vi "measure PSD Trace Values Type using CSV File.vi"(8 "error in (no error)":errorcluster, 11 "SA Measurement in":refnum<class "SA Measurement.lvclass">) -> (0 "error out":errorcluster, 3 "SA Measurement out":refnum<class "SA Measurement.lvclass">)   [LabVIEW 2023, in "Spectrum Analyzer.lvlib" / "SA Measurement.lvclass"]
uses:
  SA Measurement.lvclass
  SA Measurement.lvclass/SA Measurement.ctl
  TYPE DEFINITION/Keysight 9020A/TYPE Measurement Preset.ctl
  Spectrum Analyzer.lvlib
  TYPE DEFINITION/TYPE RBW and VBW Select.ctl
  Interface_Spectrum/Interface_Spectrum.lvclass
  TYPE DEFINITION/TYPE Marker Peak Search Type.ctl
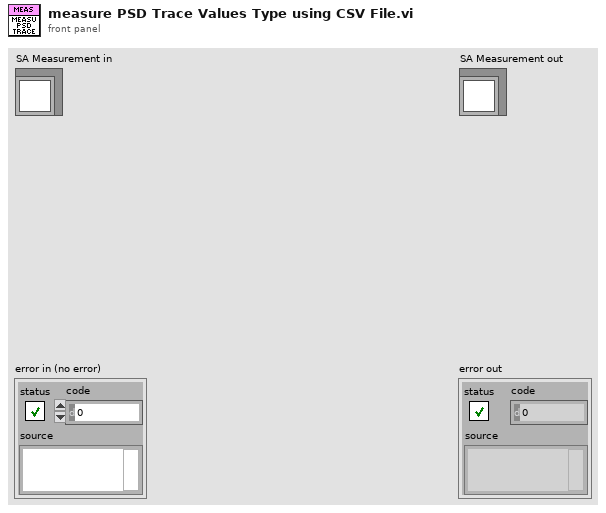
[diagram p1: front panel]
types:
  T1 = typedef "Spectrum Analyzer.lvlib/TYPE Marker Peak Search Type.ctl" = enum16{"Max", "Next Peak"}
  T2 = typedef "Spectrum Analyzer.lvlib/TYPE RBW and VBW Select.ctl" = enum16{"Res BW", "Video BW"}
  T3 = typedef "Spectrum Analyzer.lvlib/TYPE Measurement Preset.ctl" = enum16{"Sweep SA Mode", "Channel Power", "Occupied BW", "ACP", "Spurious Emission", "Spurious Emission Mask", "Burst Power (Transmit Power)"}
  T4 = typedef "Spectrum Analyzer.lvlib/TYPE Y-axis Unit.ctl" = enum16{"dBm", "dBmV", "dBuV", "dBpW", "Volt", "Ampere", "Watt"}
  T5 = typedef "Spectrum Analyzer.lvlib/TYPE Reference Level and Atten Param.ctl" = cluster{"Reference Level":dbl, "Atten":i32, "Atten Auto?":bool, "Reference Level Offset":dbl}
  T6 = typedef "Spectrum Analyzer.lvlib/TYPE Start and Stop Frequency.ctl" = cluster{"Start":dbl, "Stop":dbl}
  T7 = typedef "Spectrum Analyzer.lvlib/TYPE Display Trace Mode Select.ctl" = enum16{"Clear Write", "Max Hold", "Min Hold", "Average", "View"}
  T8 = typedef "Spectrum Analyzer.lvlib/TYPE Detect Mode Select.ctl" = enum16{"Det Auto (Normal)", "Auto Peak", "Positive Peak", "Negative Peak", "Sample", "RMS", "Average", "Quasipeak", "CISPR Average", "RMS Average"}
  T9 = cluster{"Trace Mode":T7, "Detector Type":T8, "Detect Auto?":bool}[]
  T10 = typedef "Spectrum Analyzer.lvlib/TYPE Average Mode Select.ctl" = enum16{"Linear(Voltage Avg)", "Video(Log)", "Power"}
  T11 = typedef "Spectrum Analyzer.lvlib/TYPE Marker Value.ctl" = cluster{"X-axis":dbl, "Y-axis":dbl}
  T12 = typedef "Spectrum Analyzer.lvlib/TYPE Trace Value Array.ctl" = cluster{"Frequency":dbl[], "Amplitude":dbl[]}
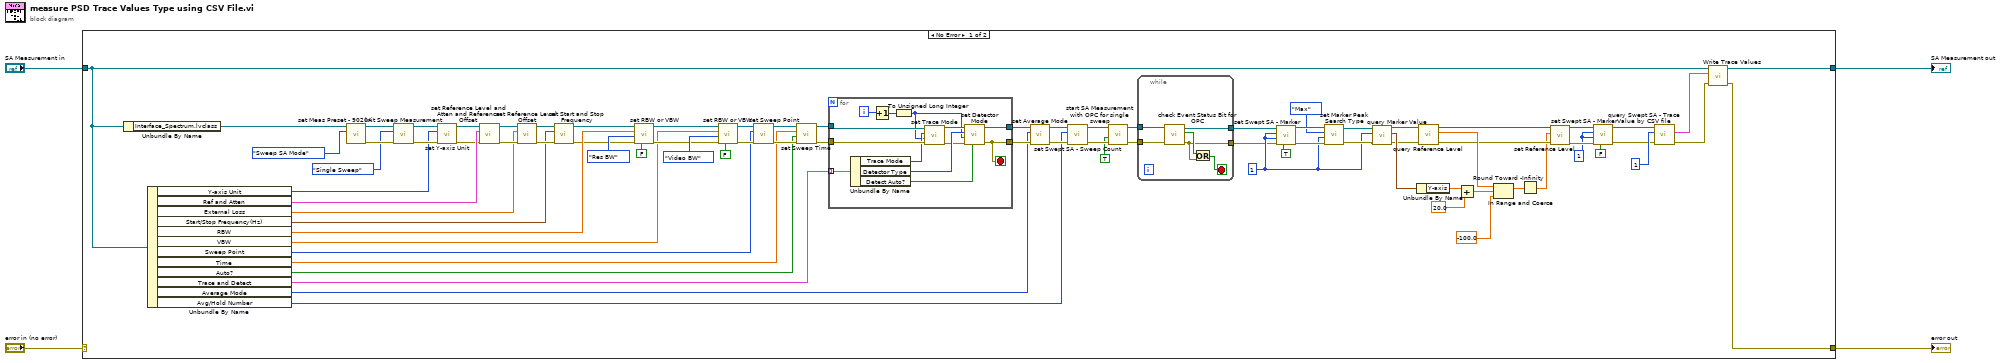
[diagram p0: block diagram]
diagram:
  n1 = case shown="No Error" "error in (no error)" {
    selector: "error in (no error)" -> [_ w106]
    tunnel: [w35 w106] -> w3
    tunnel: [w36 w105] -> w1
    tunnel: "SA Measurement in" -> [w37 w105]
    frame No Error {
      w12 = 1 ("Index")
      w28 = 1 ("Index")
      n2 = Unbundle By Name(w37) -> ("Interface_Spectrum.lvclass"=w85:refnum<class "Interface_Spectrum.lvclass">)
      n3 = Unbundle By Name(w37) -> ("Y-axis Unit"=w64:T4, "Ref and Atten"=w80:T5, "External Loss"=w77:dbl, "Start/Stop Frequency(Hz)"=w39:T6, "RBW"=w76:dbl, "VBW"=w69:dbl, "Sweep Point"=w61:u32, "Time"=w58:dbl, "Auto?"=w57:bool, "Trace and Detect"=w54:T9, "Average Mode"=w51:T10, "Avg/Hold Number"=w48:u32)
      n4 = call-dynamic "set Meas Preset - 9020A.vi"("Measurement Preset"=TYPE_Measurement_Preset."Sweep SA Mode", "Interface_Spectrum in"=w85) -> ("error out"=w82:errorcluster, "Interface_Spectrum out"=w83:refnum<class "Interface_Spectrum.lvclass">)  [unwired: 8 in]
      n5 = call-dynamic "init Sweep Measurement.vi"("error in (no error)"=w82, "Sweep Measurement Mode"=enum16{"Single Sweep", "Continuous Sweep"}."Single Sweep", "Interface_Spectrum in"=w83) -> ("error out"=w67:errorcluster, "Interface_Spectrum out"=w68:refnum<class "Interface_Spectrum.lvclass">)  [unwired: 7 in]
      n6 = call-dynamic "set Y-axis Unit.vi"("error in (no error)"=w67, "Y-axis Unit"=w64, "Interface_Spectrum in"=w68) -> ("error out"=w65:errorcluster, "Interface_Spectrum out"=w66:refnum<class "Interface_Spectrum.lvclass">)  [unwired: 7 in]
      n7 = call-dynamic "set Reference Level and Atten and Reference Offset.vi"("error in (no error)"=w65, "Reference Level, Atten, Reference Offset"=w80, "Interface_Spectrum in"=w66) -> ("error out"=w78:errorcluster, "Interface_Spectrum out"=w79:refnum<class "Interface_Spectrum.lvclass">)  [unwired: 7 in]
      n8 = call-dynamic "set Reference Level Offset.vi"("error in (no error)"=w78, "Reference Level Offset"=w77, "Interface_Spectrum in"=w79) -> ("error out"=w40:errorcluster, "Interface_Spectrum out"=w42:refnum<class "Interface_Spectrum.lvclass">)  [unwired: 7 in]
      n9 = call-dynamic "set Start and Stop Frequency.vi"("error in (no error)"=w40, "Start/Stop Frequency(Hz)"=w39, "Interface_Spectrum in"=w42) -> ("error out"=w38:errorcluster, "Interface_Spectrum out"=w41:refnum<class "Interface_Spectrum.lvclass">)  [unwired: 7 in]
      n10 = call-dynamic "set RBW or VBW.vi"("BW Auto?"=FALSE, "error in (no error)"=w38, "BW Type"=TYPE_RBW_and_VBW_Select."Res BW", "BW Value (Hz)"=w76, "Interface_Spectrum in"=w41) -> ("error out"=w70:errorcluster, "Interface_Spectrum out"=w71:refnum<class "Interface_Spectrum.lvclass">)  [unwired: 5 in]
      n11 = call-dynamic "set RBW or VBW.vi"("BW Auto?"=FALSE, "error in (no error)"=w70, "BW Type"=TYPE_RBW_and_VBW_Select."Video BW", "BW Value (Hz)"=w69, "Interface_Spectrum in"=w71) -> ("error out"=w62:errorcluster, "Interface_Spectrum out"=w63:refnum<class "Interface_Spectrum.lvclass">)  [unwired: 5 in]
      n12 = call-dynamic "set Sweep Point.vi"("error in (no error)"=w62, "Sweep Point"=w61, "Interface_Spectrum in"=w63) -> ("error out"=w59:errorcluster, "Interface_Spectrum out"=w60:refnum<class "Interface_Spectrum.lvclass">)  [unwired: 7 in]
      n13 = call-dynamic "set Sweep Time.vi"("error in (no error)"=w59, "Sweep Time Auto?"=w57, "Sweep Time(sec)"=w58, "Interface_Spectrum in"=w60) -> ("error out"=w55:errorcluster, "Interface_Spectrum out"=w56:refnum<class "Interface_Spectrum.lvclass">)  [unwired: 6 in]
      n14 = for {
        tunnel: w56 -> [w103]
        tunnel: w55 -> [w102]
        tunnel: w54 -> [w104] mode=indexing
        tunnel: [w92] -> w52
        tunnel: [w93] -> w53
        i -> [w101]
        stop <- w92 stop-if-true
        n15 = Unbundle By Name(w104) -> ("Trace Mode"=w99:T7, "Detector Type"=w97:T8, "Detect Auto?"=w94:bool)
        n16 = Increment(x=w101) -> (x+1=w100:i32)
        n17 = To Unsigned Long Integer(number=w100) -> (unsigned 32bit integer=w95:u32)
        n18 = call-dynamic "set Trace Mode.vi"("error in (no error)"=w102, "Trace Index"=w95, "Trace Mode"=w99, "Interface_Spectrum in"=w103) -> ("error out"=w96:errorcluster, "Interface_Spectrum out"=w98:refnum<class "Interface_Spectrum.lvclass">)  [unwired: 6 in]
        n19 = call-dynamic "set Detector Mode.vi"("Detect Auto?"=w94, "error in (no error)"=w96, "Trace Index"=w95, "Detector Type"=w97, "Interface_Spectrum in"=w98) -> ("error out"=w92:errorcluster, "Interface_Spectrum out"=w93:refnum<class "Interface_Spectrum.lvclass">)  [unwired: 5 in]
      }
      n20 = call-dynamic "set Average Mode.vi"("error in (no error)"=w52, "Average Mode"=w51, "Interface_Spectrum in"=w53) -> ("error out"=w49:errorcluster, "Interface_Spectrum out"=w50:refnum<class "Interface_Spectrum.lvclass">)  [unwired: 7 in]
      n21 = call-dynamic "set Swept SA - Sweep Count.vi"("error in (no error)"=w49, "Sweep Count"=w48, "Interface_Spectrum in"=w50) -> ("error out"=w46:errorcluster, "Interface_Spectrum out"=w47:refnum<class "Interface_Spectrum.lvclass">)  [unwired: 7 in]
      n22 = call-dynamic "start SA Measurement with OPC for single sweep.vi"("error in (no error)"=w46, "with OPC?"=TRUE, "Interface_Spectrum in"=w47) -> ("error out"=w43:errorcluster, "Interface_Spectrum out"=w44:refnum<class "Interface_Spectrum.lvclass">)  [unwired: 7 in]
      n23 = while {
        tunnel: w44 -> [w91]
        tunnel: w43 -> [w90]
        tunnel: [w87] -> w10
        tunnel: [w86] -> w11
        stop <- w88 stop-if-true
        n24 = call-dynamic "check Event Status Bit for OPC.vi"("error in (no error)"=w90, "Interface_Spectrum in"=w91) -> ("error out"=w87:errorcluster, "OPC Bit Changed?"=w89:bool, "Interface_Spectrum out"=w86:refnum<class "Interface_Spectrum.lvclass">)  [unwired: 7 in]
        n25 = Or(x=w89, y=w87) -> (x .or. y?=w88:bool)
      }
      n26 = call-dynamic "set Swept SA - Marker.vi"("On?"=TRUE, "error in (no error)"=w10, "trace"=w28, "Index"=w28, "Interface_Spectrum in"=w11) -> ("error out"=w32:errorcluster, "Interface_Spectrum out"=w33:refnum<class "Interface_Spectrum.lvclass">)  [unwired: 5 in]
      n27 = call-dynamic "set Marker Peak Search Type.vi"("error in (no error)"=w32, "Marker Index"=w28, "Peak Search Type"=TYPE_Marker_Peak_Search_Type."Max", "Interface_Spectrum in"=w33) -> ("error out"=w29:errorcluster, "Interface_Spectrum out"=w30:refnum<class "Interface_Spectrum.lvclass">)  [unwired: 6 in]
      n28 = call-dynamic "query Marker Value.vi"("error in (no error)"=w29, "Marker Index"=w28, "Interface_Spectrum in"=w30) -> ("error out"=w23:errorcluster, "Marker Value"=w25:T11, "Interface_Spectrum out"=w24:refnum<class "Interface_Spectrum.lvclass">)  [unwired: 6 in]
      n29 = Unbundle By Name(w25) -> ("Y-axis"=w27:dbl)
      n30 = call-dynamic "query Reference Level.vi"("error in (no error)"=w23, "Interface_Spectrum in"=w24) -> ("error out"=w18:errorcluster, "Ref Level"=w21:dbl, "Interface_Spectrum out"=w22:refnum<class "Interface_Spectrum.lvclass">)  [unwired: 7 in]
      n31 = Add(x=w27, y=20.0) -> (x+y=w20:dbl)
      n32 = In Range and Coerce(upper limit=w21, x=w20, lower limit=-100.0) -> (coerced(x)=w17:dbl)  [unwired: 1 out]
      n33 = Round Toward -Infinity(1:w17) -> (0:w16:dbl)
      n34 = call-dynamic "set Reference Level.vi"("error in (no error)"=w18, "Reference Level"=w16, "Interface_Spectrum in"=w22) -> ("error out"=w14:errorcluster, "Interface_Spectrum out"=w15:refnum<class "Interface_Spectrum.lvclass">)  [unwired: 7 in]
      n35 = call-dynamic "set Swept SA - Marker.vi"("On?"=FALSE, "error in (no error)"=w14, "trace"=w12, "Index"=w12, "Interface_Spectrum in"=w15) -> ("error out"=w7:errorcluster, "Interface_Spectrum out"=w9:refnum<class "Interface_Spectrum.lvclass">)  [unwired: 5 in]
      n36 = call-dynamic "query Swept SA - Trace Value by CSV file.vi"("error in (no error)"=w7, "Trace Index"=u32 1, "Interface_Spectrum in"=w9) -> ("error out"=w5:errorcluster, "Trace Values"=w6:T12)  [unwired: 6 in, 1 out]
      n37 = call "Write Trace Values.vi"("error in (no error)"=w5, "Trace Values"=w6, "SA Measurement in"=w37) -> ("error out"=w35:errorcluster, "SA Measurement out"=w36:refnum<class "SA Measurement.lvclass">)  [unwired: 7 in]
    }
    frame Error {
    }
  }
  "error out" <- w3
  "SA Measurement out" <- w1
